vi "PicoScope6000aOpen.vi"(5 "Serial Number":string, 7 "Use Serial Number":bool, 8 "error in (no error)":errorcluster, 9 "Mode":u16(ring) items=["Dialog On Error", "no dialog - CloseUnit and Stop", "no dialog - Continue", "no dialog - Stop"], 10 "Resolution":u32(ring) items=["8-bit"=0, "12-bit"=1, "14-bit"=2, "15-bit"=3, "16-bit"=4, "10-bit"=10]) -> (0 "error out":errorcluster, 1 "Max ADC value":i16, 2 "Device Info":T1, 3 "handle out":i16, 4 "Pico 6000a Units":string, 6 "serialLth":i16)   [LabVIEW 2010]
doc: "This VI manages listing and opens devices with device details."
uses:
  ps6000a.dll
panel:
  out "minValue":i16
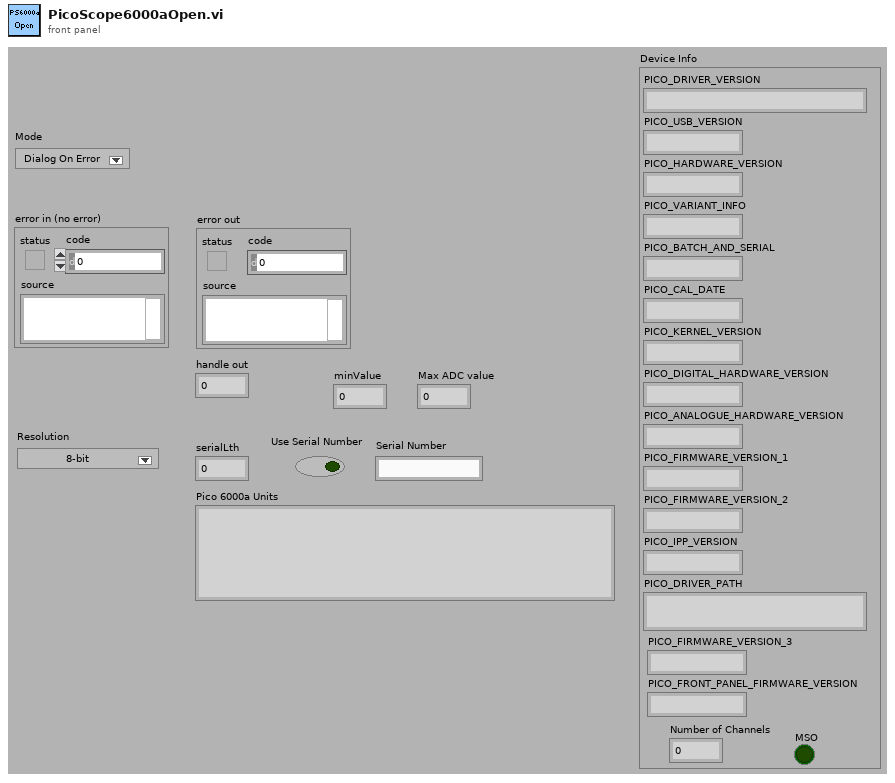
[diagram p1: front panel]
types:
  T1 = cluster{"PICO_DRIVER_VERSION":string, "PICO_USB_VERSION":string, "PICO_HARDWARE_VERSION":string, "PICO_VARIANT_INFO":string, "PICO_BATCH_AND_SERIAL":string, "PICO_CAL_DATE":string, "PICO_KERNEL_VERSION":string, "PICO_DIGITAL_HARDWARE_VERSION":string, "PICO_ANALOGUE_HARDWARE_VERSION":string, "PICO_FIRMWARE_VERSION_1":string, "PICO_FIRMWARE_VERSION_2":string, "PICO_IPP_VERSION":string, "PICO_DRIVER_PATH":string, "PICO_FIRMWARE_VERSION_3":string, "PICO_FRONT_PANEL_FIRMWARE_VERSION":string, "Number of Channels":i16, "MSO":bool}
  T2 = cluster{"status":bool, "code":u32, "source":string}
  T3 = cluster{"PICO_DRIVER_VERSION":string, "PICO_USB_VERSION":string, "PICO_HARDWARE_VERSION":string, "PICO_VARIANT_INFO":string, "PICO_BATCH_AND_SERIAL":string, "PICO_CAL_DATE":string, "PICO_KERNEL_VERSION":string, "PICO_DIGITAL_HARDWARE_VERSION":string, "PICO_ANALOGUE_HARDWARE_VERSION":string, "PICO_FIRMWARE_VERSION_1":string, "PICO_FIRMWARE_VERSION_2":string, "PICO_IPP_VERSION":string, "PICO_DRIVER_PATH":string, "PICO_FIRMWARE_VERSION_3":string, "PICO_FRONT_PANEL_FIRMWARE_VERSION":string}
  T4 = cluster{"PICO_DRIVER_VERSION":string, "PICO_USB_VERSION":string, "PICO_HARDWARE_VERSION":string, "PICO_VARIANT_INFO":string, "PICO_BATCH_AND_SERIAL":string, "PICO_CAL_DATE":string, "PICO_KERNEL_VERSION":string, "PICO_DIGITAL_HARDWARE_VERSION":string, "PICO_ANALOGUE_HARDWARE_VERSION":string, "PICO_FIRMWARE_VERSION_1":string, "PICO_FIRMWARE_VERSION_2":string, "PICO_IPP_VERSION":string, "PICO_DRIVER_PATH":string, "PICO_FIRMWARE_VERSION_3":string, "PICO_FRONT_PANEL_FIRMWARE_VERSION":string, i16, "x != y?":bool}
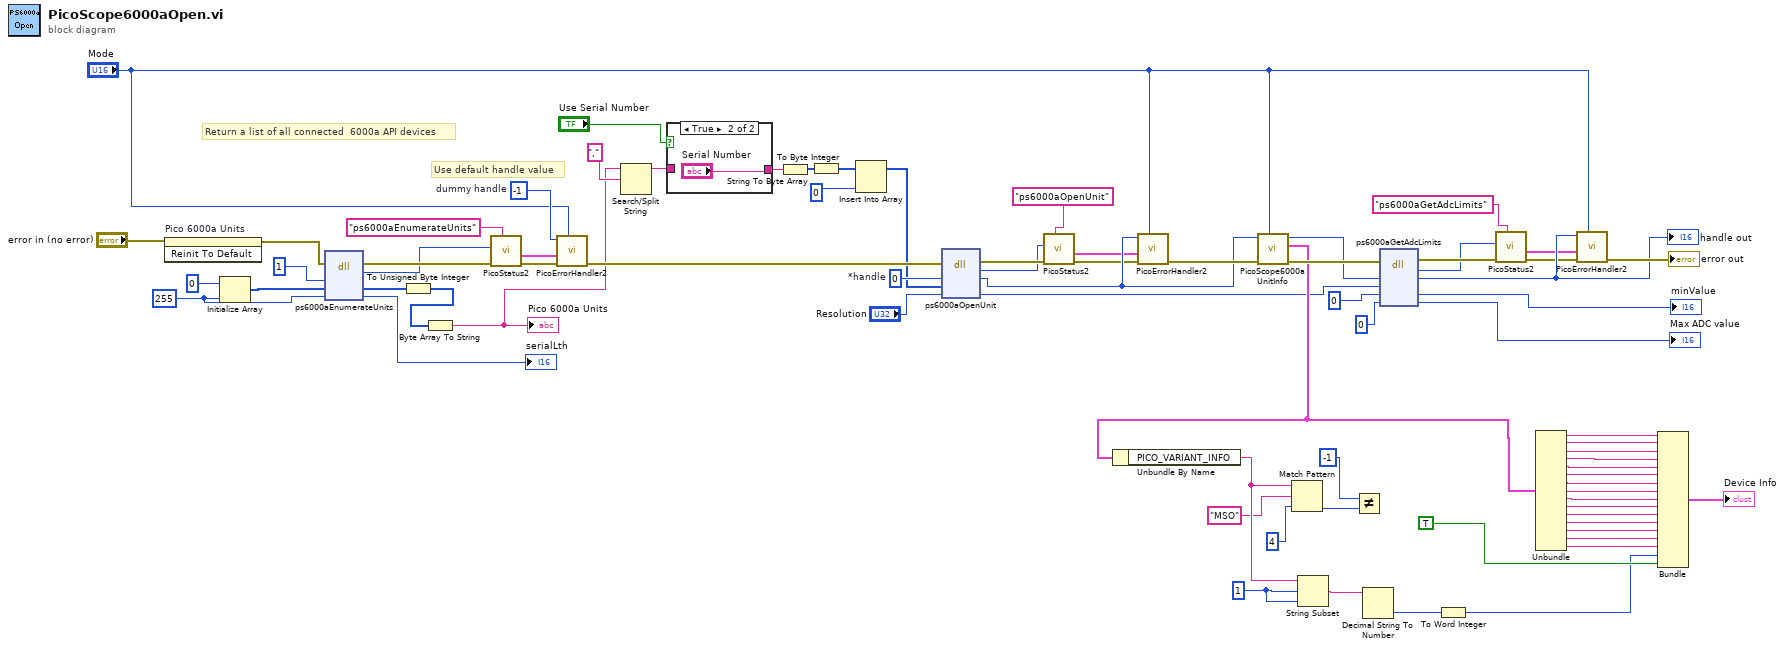
[diagram p0: block diagram]
diagram:
  w27 = i16 -1  # dummy handle
  w31 = i16 255 ("dimension size")
  w66 = 1 ("offset (0)")
  w39 = i16 0  # *handle
  # "Use default handle value"
  # "Return a list of all connected  6000a API devices"
  n1 = invoke on="Pico 6000a Units" class="Str" method="Reinit To Default"(error in="error in (no error)") -> (error out=w28:errorcluster)  [unwired: 2 in, 2 out]
  n2 = Initialize Array(i8 0 ("U8"), w31) -> (w33:i8[])
  n3 = dll-call lib="ps6000a.dll" fn="ps6000aEnumerateUnits"(error in=w28, "count"=i16 1, "serials"=w33, "serialLth"=w31) -> (error out=w24:errorcluster, "PICO_STATUS"=w21:u32, "serials"=w29:i8[], "serialLth"=→"serialLth":i16)  [unwired: 3 in, 1 out]
  n4 = To Unsigned Byte Integer(number=w29) -> (unsigned 8bit integer=w30:u8[])
  n5 = Byte Array To String(unsigned byte array=w30) -> (string=w14:string)
  "Pico 6000a Units" <- w14
  n6 = call "PicoStatus2.vi"("PICO source"="ps6000aEnumerateUnits" ("source"), "Error in"=w24, "PICO STATUS"=w21) -> ("error out"=w25:errorcluster, "PICO_STATUS out"=w23:T2)  [unwired: 5 in]
  n7 = call "PicoErrorHandler2.vi"("Mode"="Mode", "error in (no error)"=w25, "PICO_STATUS in"=w23, "handle In"=w27) -> ("error out"=w38:errorcluster)  [unwired: 7 in]
  n8 = Search/Split String(string=w14, search string/char (-)=",") -> (substring before match=w19:string)  [unwired: 1 in, 2 out]
  n9 = case shown="True" "Use Serial Number" {
    tunnel: w19 -> [w77 _]
    tunnel: [w77 "Serial Number"] -> w15
    frame False {
    }
    frame True {
    }
  }
  n10 = String To Byte Array(string=w15) -> (unsigned byte array=w17:u8[])
  n11 = To Byte Integer(number=w17) -> (8bit integer=w18:i8[])
  n12 = Insert Into Array(array=w18, new element=i8 0 ("new element/subarray")) -> (w12:i8[])  [unwired: 1 in]
  n13 = dll-call lib="ps6000a.dll" fn="ps6000aOpenUnit" ("ps3000.dll:_ps3000_open_unit@0")(error in=w38, "handle"=w39, "serial"=w12, "resolution"="Resolution") -> (error out=w10:errorcluster, "PICO_STATUS"=w2:u32, "handle"=w26:i16, "resolution"=w36:u32)  [unwired: 3 in, 1 out]
  n14 = call "PicoStatus2.vi"("PICO source"="ps6000aOpenUnit" ("source"), "Error in"=w10, "PICO STATUS"=w2) -> ("error out"=w11:errorcluster, "PICO_STATUS out"=w5:T2)  [unwired: 5 in]
  n15 = call "PicoErrorHandler2.vi"("Mode"="Mode", "error in (no error)"=w11, "PICO_STATUS in"=w5, "handle In"=w26) -> ("error out"=w76:errorcluster)  [unwired: 7 in]
  n16 = call "PicoScope6000aUnitInfo.vi"("Mode"="Mode", "error in (no error)"=w76, "handle in"=w26) -> ("error out"=w59:errorcluster, "Unit Info"=w52:T3, "handle out"=w57:i16)  [unwired: 6 in]
  n17 = Unbundle By Name(w52) -> ("PICO_VARIANT_INFO"=w65:string)
  n18 = Match Pattern(string=w65, regular expression="MSO", offset (0)=4) -> (offset past match=w62:i32)  [unwired: 3 out]
  n19 = String Subset(string=w65, offset (0)=w66, length (rest)=w66) -> (substring=w45:string)
  n20 = Not Equal?(x=-1, y=w62) -> ()  [unwired: 1 out]
  n21 = Decimal String To Number(string=w45) -> (number=w41:i32)  [unwired: 2 in, 1 out]
  n22 = dll-call lib="ps6000a.dll" fn="ps6000aGetAdcLimits" ("ps3000.dll:_ps3000_open_unit@0")(error in=w59, "handle"=w57, "resolution"=w36, "minValue"=i16 0, "maxValue"=i16 0 ("manValue")) -> (error out=w8:errorcluster, "PICO_STATUS"=w3:u32, "handle"=w58:i16, "minValue"=→"minValue":i16, "maxValue"=→"Max ADC value":i16)  [unwired: 3 in, 1 out]
  "handle out" <- w58
  n23 = To Word Integer(number=w41) -> (16bit integer=w40:i16)
  n24 = call "PicoStatus2.vi"("PICO source"="ps6000aGetAdcLimits" ("source"), "Error in"=w8, "PICO STATUS"=w3) -> ("error out"=w9:errorcluster, "PICO_STATUS out"=w7:T2)  [unwired: 5 in]
  n25 = Unbundle(w52) -> ("PICO_DRIVER_VERSION"=w75:string, "PICO_USB_VERSION"=w74:string, "PICO_HARDWARE_VERSION"=w73:string, "PICO_VARIANT_INFO"=w72:string, "PICO_BATCH_AND_SERIAL"=w71:string, "PICO_CAL_DATE"=w70:string, "PICO_KERNEL_VERSION"=w69:string, "PICO_DIGITAL_HARDWARE_VERSION"=w68:string, "PICO_ANALOGUE_HARDWARE_VERSION"=w67:string, "PICO_FIRMWARE_VERSION_1"=w51:string, "PICO_FIRMWARE_VERSION_2"=w50:string, "PICO_IPP_VERSION"=w49:string, "PICO_DRIVER_PATH"=w48:string, "PICO_FIRMWARE_VERSION_3"=w47:string, "PICO_FRONT_PANEL_FIRMWARE_VERSION"=w46:string)
  n26 = call "PicoErrorHandler2.vi"("Mode"="Mode", "error in (no error)"=w9, "PICO_STATUS in"=w7, "handle In"=w58) -> ("error out"=→"error out":errorcluster)  [unwired: 7 in]
  n27 = Bundle("PICO_DRIVER_VERSION"=w75, "PICO_USB_VERSION"=w74, "PICO_HARDWARE_VERSION"=w73, "PICO_VARIANT_INFO"=w72, "PICO_BATCH_AND_SERIAL"=w71, "PICO_CAL_DATE"=w70, "PICO_KERNEL_VERSION"=w69, "PICO_DIGITAL_HARDWARE_VERSION"=w68, "PICO_ANALOGUE_HARDWARE_VERSION"=w67, "PICO_FIRMWARE_VERSION_1"=w51, "PICO_FIRMWARE_VERSION_2"=w50, "PICO_IPP_VERSION"=w49, "PICO_DRIVER_PATH"=w48, "PICO_FIRMWARE_VERSION_3"=w47, "PICO_FRONT_PANEL_FIRMWARE_VERSION"=w46, w40, "x != y?"=TRUE) -> (→"Device Info":T4)  [unwired: 1 in]
